vi "Generate Filename.vi"(8 "error in":errorcluster, 10 "Folder":path, 11 "LabVIEW File in":refnum<class "LabVIEW File.lvclass">) -> (0 "error out":errorcluster, 2 "File Path":path, 3 "LabVIEW File out":refnum<class "LabVIEW File.lvclass">)   [LabVIEW 2026, in "LabVIEW File.lvclass"]
doc: "This VI generates a file path suitable for saving files based on the provided folder and the implementing classes properties."
uses:
  LabVIEW File.lvclass
  LabVIEW File.lvclass/LabVIEW File.ctl
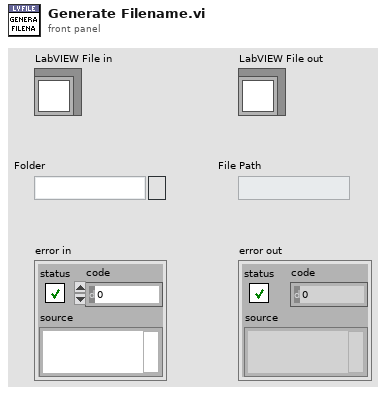
[diagram p1: front panel]
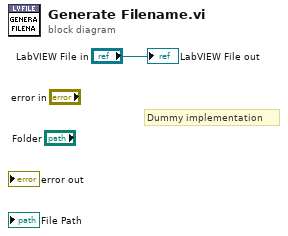
[diagram p0: block diagram]
diagram:
  # "Dummy implementation"
  "LabVIEW File out" <- "LabVIEW File in"
